vi "Adjust FIFO Size.vi"(8 "error in (no error)":errorcluster, 10 "New FIFO Instance Config":T1 {"Custom Data" format="%.0x"}, 11 "CIF_CIPC_Chn in":refnum<class "CIF_Iceoryx_Chn.lvclass">) -> (0 "error out":errorcluster, 3 "CIF_CIPC_Chn out":refnum<class "CIF_Iceoryx_Chn.lvclass">)   [LabVIEW 2021, in "CIF_Iceoryx_Chn.lvclass"]
uses:
  CIF_Iceoryx_Chn.lvclass
  ChannelCommon/typedef/New FIFO Instance Configuration.ctl
  CIF_Iceoryx_Chn.lvclass/CIF_Iceoryx_Chn.ctl
  ChannelCommon/ChannelCommon.lvlib
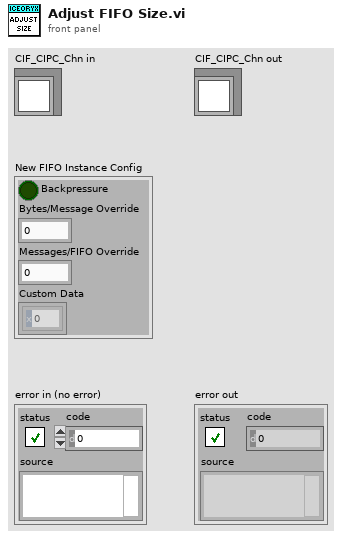
[diagram p1: front panel]
types:
  T1 = typedef "ChannelCommon.lvlib/New FIFO Instance Configuration.ctl" = cluster{"Backpressure":bool, "Bytes/Message Override":u32, "Messages/FIFO Override":u32, "Custom Data":u8[]}
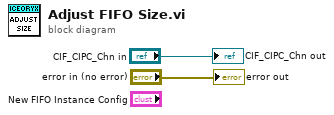
[diagram p0: block diagram]
diagram:
  "error out" <- "error in (no error)"
  "CIF_CIPC_Chn out" <- "CIF_CIPC_Chn in"
